vi "Watchdog Acknowledge.vi"(4 "error in (no error)":errorcluster, 7 "watchdogID in":u64 format="%.0x") -> (0 "error out":errorcluster, 1 "watchdog status":T1, 3 "watchdogID out":u64 format="%.0x")   [LabVIEW 2025]
doc: "<p>Resets the <a href=\"nihelplauncher://docs/csh?context=lvrt_lvrtconcepts_rt_watchdog\">watchdog counter</a> to the specified count, but does not start the countdown if the counter has not yet started or has expired.</p>"
uses:
  niwd4c.dll
  Watchdog status enum.ctl
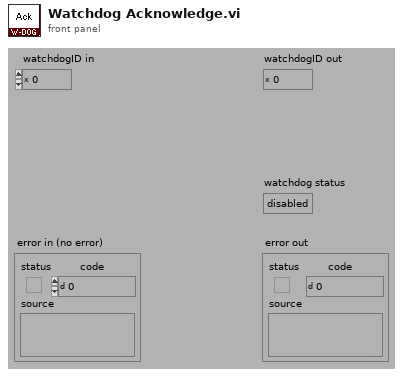
[diagram p1: front panel]
types:
  T1 = typedef "Watchdog status enum.ctl" = enum16{"disabled", "expired", "running"}
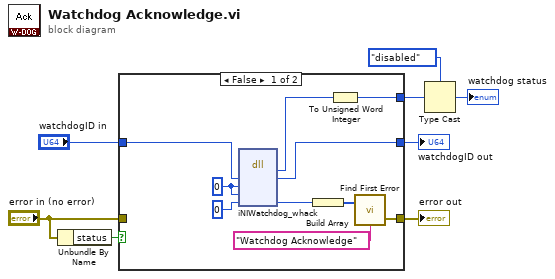
[diagram p0: block diagram]
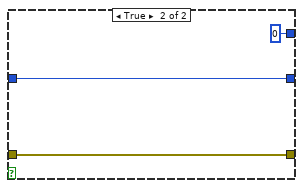
[diagram p2: hidden frame]
diagram:
  n1 = Unbundle By Name("error in (no error)") -> ("status"=w8:bool)
  n2 = case shown="False" w8 {
    tunnel: [w15 w20] -> w5
    tunnel: [w17 w21] -> w4
    tunnel: "error in (no error)" -> [_ w21]
    tunnel: "watchdogID in" -> [w14 w20]
    tunnel: [w10 u16 0] -> w3
    frame False {
      w9 = u32 0 ("currentCount")
      n3 = dll-call lib="niwd4c.*" fn="iNIWatchdog_whack" label="Whack"("wd"=w14, "newInitialCount"=w9, "currentCount"=w9, "status"=0) -> ("return type"=w11:u32, "wd"=w15:u64, "status"=w13:i32)  [unwired: 5 in, 2 out]
      n4 = Build Array(w13) -> (w18:i32[])
      n5 = To Unsigned Word Integer(number=w11) -> (unsigned 16bit integer=w10:u16)
      n6 = call <vilib>:"Find First Error.vi"("source messages"="Watchdog Acknowledge", "error codes"=w18) -> ("error out"=w17:errorcluster)  [unwired: 2 in, 1 out]
    }
    frame True {
    }
  }
  "error out" <- w4
  "watchdogID out" <- w5
  n7 = Type Cast(type=enum16{"disabled", "expired", "running"}."disabled" ("watchdog status"), x=w3) -> (*(type *) &x=→"watchdog status":enum16{"disabled", "expired", "running"})
